vi "GOOPUtil_GetClassMembers.vi"(0 "LVClassPath":path, 5 "error in (no error)":errorcluster) -> (14 "MemberPaths":T1[](array[typedef]), 19 "error out":errorcluster)   [LabVIEW 2020, in "GOOPUtility.lvlib"]
doc: "Returns all class members paths, names and scopes (except the util VIs) from a given GOOP class path.\n\nNote: This will not work if the .lvclass file is inside an .exe file.\n\nThis is a collection of generic GOOP utility VIs. Please notice that it is important that the frontpanel of the Create, Destroy and GetObjectStatus is not removed when building an application."
uses:
  GOOPUtility.lvlib
  GOOPUtil_MemberDefinition.ctl
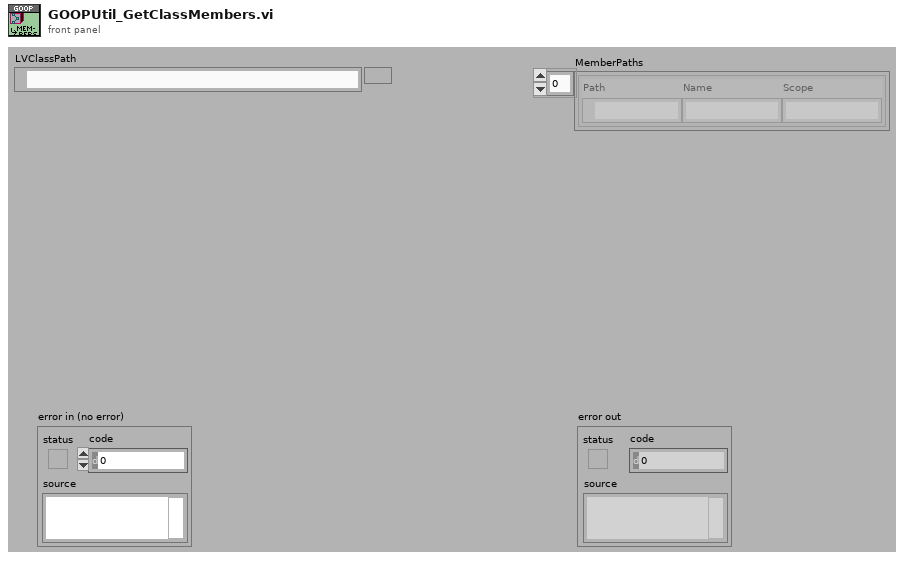
[diagram p1: front panel]
types:
  T1 = typedef "GOOPUtility.lvlib/GOOPUtil_MemberDefinition.ctl" = cluster{"Path":path, "Name":string, "Scope":string}
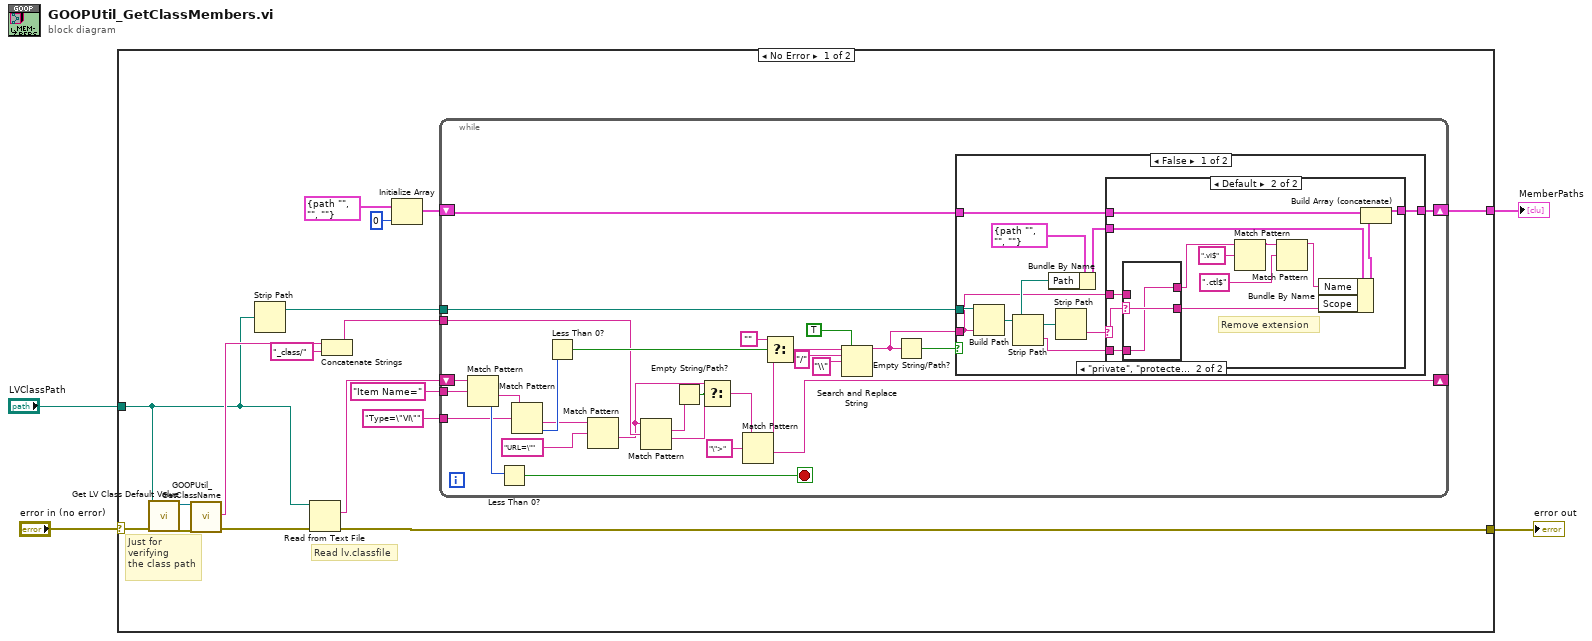
[diagram p0: block diagram]
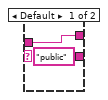
[diagram p3: hidden frame]
diagram:
  n1 = case shown="No Error" "error in (no error)" {
    selector: "error in (no error)" -> [w18 w80]
    tunnel: [w6 w80] -> w3
    tunnel: "LVClassPath" -> [w5 _]
    tunnel: [w16 _] -> w1
    frame No Error {
      # "Read lv.classfile"
      # "Just for\nverifying\nthe class path"
      n2 = call <vilib>:"Get LV Class Default Value.vi"("error in (no error)"=w18, "class path"=w5) -> ("error out"=w12:errorcluster, "object"=w11:refnum<class>)  [unwired: 8 in]
      n3 = call "GOOPUtil_GetClassName.vi"("LabVIEW Object"=w11, "error in (no error)"=w12) -> ("Class Name"=w10:string, "error out"=w7:errorcluster)  [unwired: 13 in, 3 out]
      n4 = Strip Path(path=w5) -> (stripped path=w17:path)  [unwired: 1 out]
      n5 = Read from Text File(file (use dialog)=w5, error in=w7) -> (text=w19:string, error out=w6:errorcluster)  [unwired: 1 in, 3 out]
      n6 = Concatenate Strings(w10, "_class/" ("string")) -> (w8:string)
      n7 = Initialize Array(T1 {"Path"=path "", "Name"="", "Scope"=""} ("Member"), 0 ("dimension size")) -> (w15:T1[])
      n8 = while {
        shift-right: [w37] -> _
        shift-left: w19 -> [w50]
        tunnel: "Item Name=" ("Search Tag") -> [w46]
        tunnel: "Type=\"VI\"" ("regular expression") -> [w45]
        shift-right: [w28] -> w16
        shift-left: w15 -> [w31]
        tunnel: w17 -> [w30]
        tunnel: w8 -> [w27]
        stop <- w47 stop-if-true
        n9 = Match Pattern(string=w50, regular expression=w46) -> (after substring=w49:string, offset past match=w48:i32)  [unwired: 3 out]
        n10 = Less Than 0?(x=w48) -> (x < 0?=w47:bool)
        n11 = Match Pattern(string=w49, regular expression=w45) -> (after substring=w41:string, offset past match=w44:i32)  [unwired: 3 out]
        n12 = Less Than 0?(x=w44) -> (x < 0?=w42:bool)
        n13 = Match Pattern(string=w41, regular expression="URL=\"" ("search string/char (-)")) -> (after substring=w24:string)  [unwired: 4 out]
        n14 = Match Pattern(string=w24, regular expression=w27) -> (match substring=w26:string, after substring=w23:string)  [unwired: 3 out]
        n15 = Empty String/Path?(string/path=w26) -> (empty?=w25:bool)
        n16 = Select(t=w24, s=w25, f=w23) -> (s? t:f=w22:string)
        n17 = Match Pattern(string=w22, regular expression="\">" ("search string/char (-)")) -> (before substring=w38:string, after substring=w37:string)  [unwired: 3 out]
        n18 = Select(t="", s=w42, f=w38) -> (s? t:f=w36:string)
        n19 = Search and Replace String(replace all?=TRUE ("replace all? (F)"), input string=w36, search string="/" ("search string/char (-)"), replace string="\\" ("search string/char (-)")) -> (result string=w29:string)  [unwired: 1 in, 6 out]
        n20 = Empty String/Path?(string/path=w29) -> (empty?=w32:bool)
        n21 = case shown="False" w32 {
          tunnel: w31 -> [w60 w79]
          tunnel: w30 -> [w59 _]
          tunnel: w29 -> [w52 _]
          tunnel: [w58 w79] -> w28
          frame False {
            n22 = Build Path(base path=w59, name or relative path=w52) -> (appended path=w54:path)
            n23 = Strip Path(path=w54) -> (stripped path=w57:path, name=w51:string)
            n24 = Bundle By Name(cluster=T1 {"Path"=path "", "Name"="", "Scope"=""} ("Member"), "Path"=w54) -> (w53:T1)
            n25 = Strip Path(path=w57) -> (name=w56:string)  [unwired: 1 out]
            n26 = case shown="Default" w56 {
              selector: w56 -> [_ w70]
              tunnel: w60 -> [w61 w74]
              tunnel: [w61 w71] -> w58
              tunnel: w53 -> [_ w73]
              tunnel: w52 -> [_ w68]
              tunnel: w51 -> [_ w67]
              frame "utils" {
                # "Don't include the utils VIs that is only for\nthe GOOP implementation."
              }
              frame Default {
                # "Remove extension"
                n27 = case shown="\"private\", \"protected\"" w70 {
                  selector: w70 -> [_ w78]
                  tunnel: ["public" w78] -> w69
                  tunnel: w68 -> [w75 _]
                  tunnel: w67 -> [_ w77]
                  tunnel: [w75 w77] -> w65
                  frame Default {
                  }
                  frame "private", "protected" {
                  }
                }
                n28 = Match Pattern(string=w65, regular expression=".vi$") -> (before substring=w64:string)  [unwired: 1 in, 3 out]
                n29 = Match Pattern(string=w64, regular expression=".ctl$") -> (before substring=w63:string)  [unwired: 1 in, 3 out]
                n30 = Bundle By Name(cluster=w73, "Name"=w63, "Scope"=w69) -> (w72:T1)
                n31 = Build Array (concatenate)(w74, w72) -> (w71:T1[])
              }
            }
          }
          frame True {
            # "False alarm..."
          }
        }
      }
    }
    frame Error {
    }
  }
  "error out" <- w3
  "MemberPaths" <- w1
